vi "C_Echo_RT.vi"(0 "tx in":u8[](array[numeric]), 1 "flags":u16[](array[numeric]), 2 "data len":u8[](array[numeric]), 3 "data":u8[](array[numeric]), 5 "new id":u32, 7 "index":i32, 9 "n frames":i32, 11 "error in (no error)":errorcluster) -> (4 "tx out":u8[](array[numeric]), 6 "length":i32, 15 "error out":errorcluster)   [LabVIEW 2021, in "CANsub_C.lvlib"]
doc: "Real-time echo: encodes received frame number index with a new ID (IDE, FDF, BRS and data kept) into the caller’s tx buffer. No allocation. Send tx bytes 0 … length - 1. Error frames and index = n frames give an error."
uses:
  CANsub_C.lvlib
  codec_vis/CANsub_Codec.lvlib
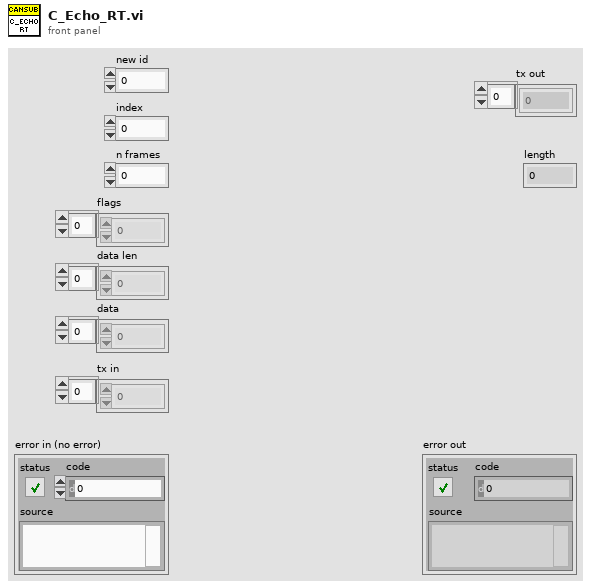
[diagram p1: front panel]
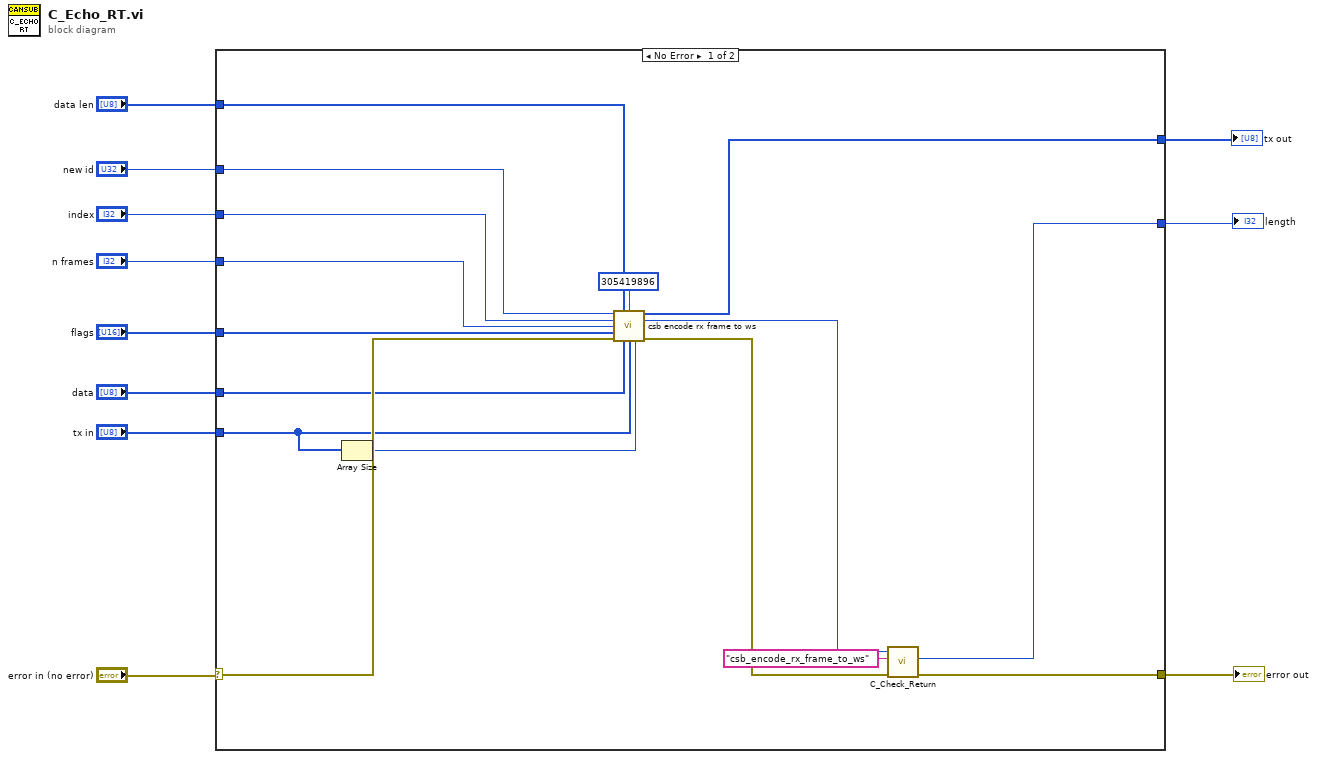
[diagram p0: block diagram]
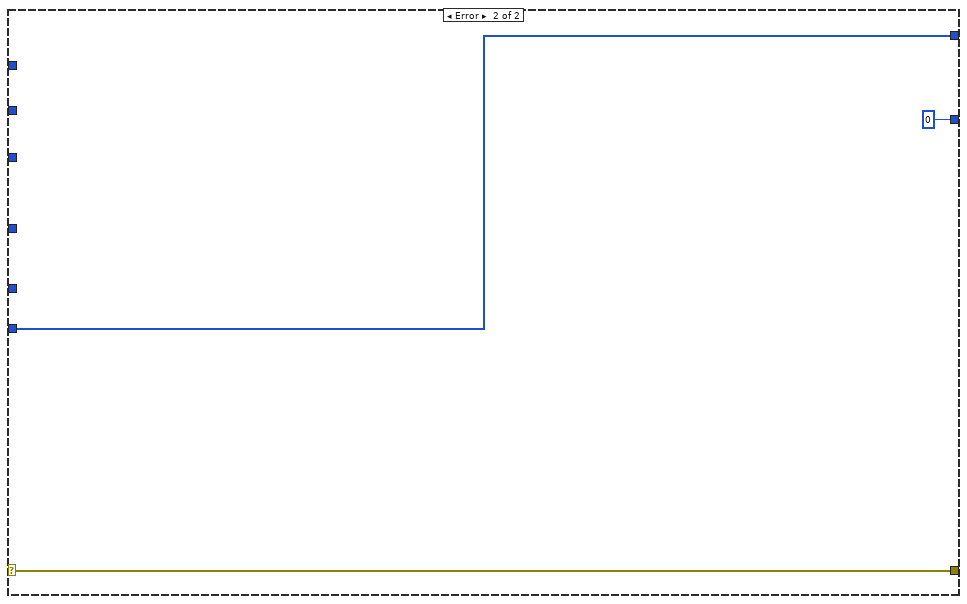
[diagram p2: hidden frame]
diagram:
  n1 = case shown="No Error" "error in (no error)" {
    selector: "error in (no error)" -> [w26 w28]
    tunnel: [w25 w28] -> w10
    tunnel: [w15 w30] -> w9
    tunnel: "tx in" -> [w16 w30]
    tunnel: [w13 0 ("length")] -> w7
    tunnel: "new id" -> [w24 _]
    tunnel: "index" -> [w23 _]
    tunnel: "n frames" -> [w22 _]
    tunnel: "flags" -> [w21 _]
    tunnel: "data" -> [w20 _]
    tunnel: "data len" -> [w19 _]
    frame No Error {
      n2 = Array Size(array=w16) -> (size(s)=w17:i32)
      n3 = call "csb encode rx frame to ws.vi"("new_id"=w24, "data_len"=w19, "mask"=u32 305419896, "out_cap"=w17, "index"=w23, "n_frames"=w22, "flags"=w21, "error in (no error)"=w26, "data"=w20, "out"=w16) -> ("out out"=w15:u8[], "function return"=w14:i32, "error out"=w27:errorcluster)  [unwired: 3 in]
      n4 = call "C_Check_Return.vi"("error in (no error)"=w27, "function name"="csb_encode_rx_frame_to_ws", "function return"=w14) -> ("error out"=w25:errorcluster, "length"=w13:i32)  [unwired: 6 in, 1 out]
    }
    frame Error {
    }
  }
  "error out" <- w10
  "tx out" <- w9
  "length" <- w7
